vi "RunVI.vi"(0 "VI Reference In":refnum<vi>, 5 "Wait Until Done (F)":bool, 7 "Auto Dispose Reference (F)":bool, 9 "Ignore If Already Running (T)":bool=TRUE, 11 "error in":errorcluster) -> (4 "VI Reference Out":refnum<vi>, 15 "error out":errorcluster)   [LabVIEW 2016, in "Drona.lvlib" / "VI.lvlib"]
doc: "Runs the specified VI."
uses:
  VI.lvlib
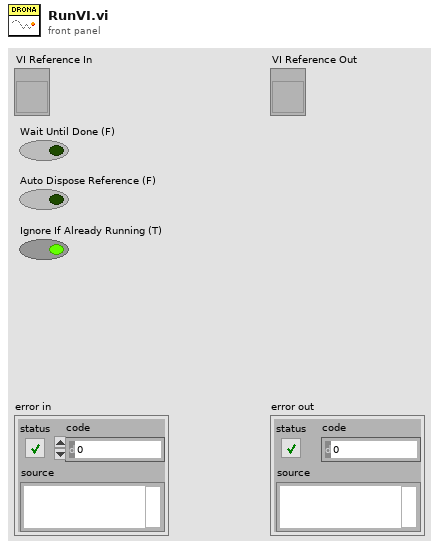
[diagram p1: front panel]
types:
  T1 = enum32{"Bad", "Idle", "Run top level", "Running"}
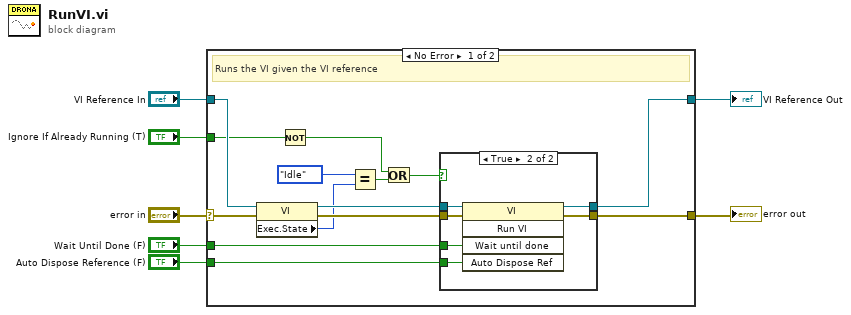
[diagram p0: block diagram]
diagram:
  n1 = case shown="No Error" "error in" {
    selector: "error in" -> [w17 w31]
    tunnel: "VI Reference In" -> [w15 w30]
    tunnel: [w20 w30] -> w5
    tunnel: [w21 w31] -> w4
    tunnel: "Wait Until Done (F)" -> [w19 _]
    tunnel: "Auto Dispose Reference (F)" -> [w18 _]
    tunnel: "Ignore If Already Running (T)" -> [w10 _]
    frame No Error {
      # "Runs the VI given the VI reference"
      n2 = property class="VI"(reference=w15, error in=w17) -> (reference out=w14:refnum<vi>, error out=w16:errorcluster, "Exec.State"=w13:T1)
      n3 = Not(x=w10) -> (.not. x?=w8:bool)
      n4 = Equal?(x=T1."Idle", y=w13) -> (x = y?=w11:bool)
      n5 = Or(x=w8, y=w11) -> (x .or. y?=w9:bool)
      n6 = case shown="True" w9 {
        tunnel: [w23 w29] -> w21
        tunnel: [w22 w28] -> w20
        tunnel: w19 -> [_ w27]
        tunnel: w18 -> [_ w26]
        tunnel: w16 -> [w23 w25]
        tunnel: w14 -> [w22 w24]
        frame False {
        }
        frame True {
          n7 = invoke on="Invoke Node" class="VI" method="Run VI"(reference=w24, error in=w25, "Wait until done"=w27, "Auto Dispose Ref"=w26) -> (reference out=w28:refnum<vi>, error out=w29:errorcluster)  [unwired: 1 in, 3 out]
        }
      }
    }
    frame Error {
    }
  }
  "error out" <- w4
  "VI Reference Out" <- w5
